vi "query UL_DL Channel Bandwidth.vi"(8 "error in (no error)":errorcluster, 9 "Direction":T1, 10 "Bandwidth Setting Param":T2, 11 "NR in":refnum<class "NR.lvclass">) -> (0 "error out":errorcluster, 2 "BW (MHz)":u32, 3 "NR out":refnum<class "NR.lvclass">)   [LabVIEW 2023, in "ANRITSU Call Box.lvlib" / "NR.lvclass"]
uses:
  NR.lvclass
  NR.lvclass/NR.ctl
  Type Definition/Uplink Downlink Enum.ctl
  ANRITSU Call Box.lvlib
  Type Definition/NR Channel Bandwidth Param.ctl
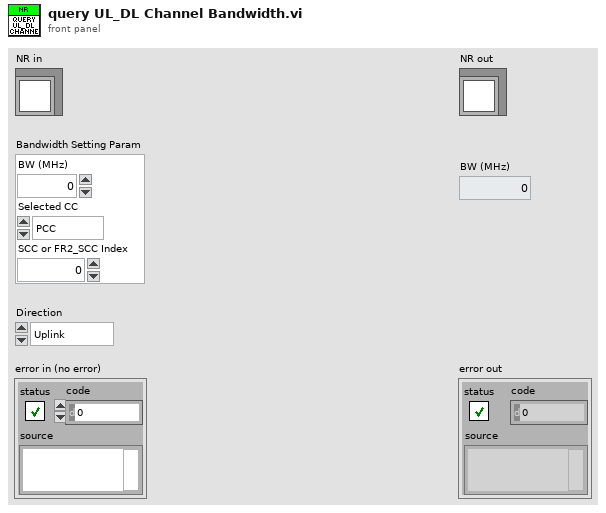
[diagram p1: front panel]
types:
  T1 = typedef "ANRITSU Call Box.lvlib/Uplink Downlink Enum.ctl" = enum16{"Uplink", "Downlink"}
  T2 = typedef "ANRITSU Call Box.lvlib/NR Channel Bandwidth Param.ctl" = cluster{"BW (MHz)":u32, "Selected CC":enum16{"PCC", "SCC", "FR2_PCC", "FR2_SCC"}, "SCC or FR2_SCC Index":u32}
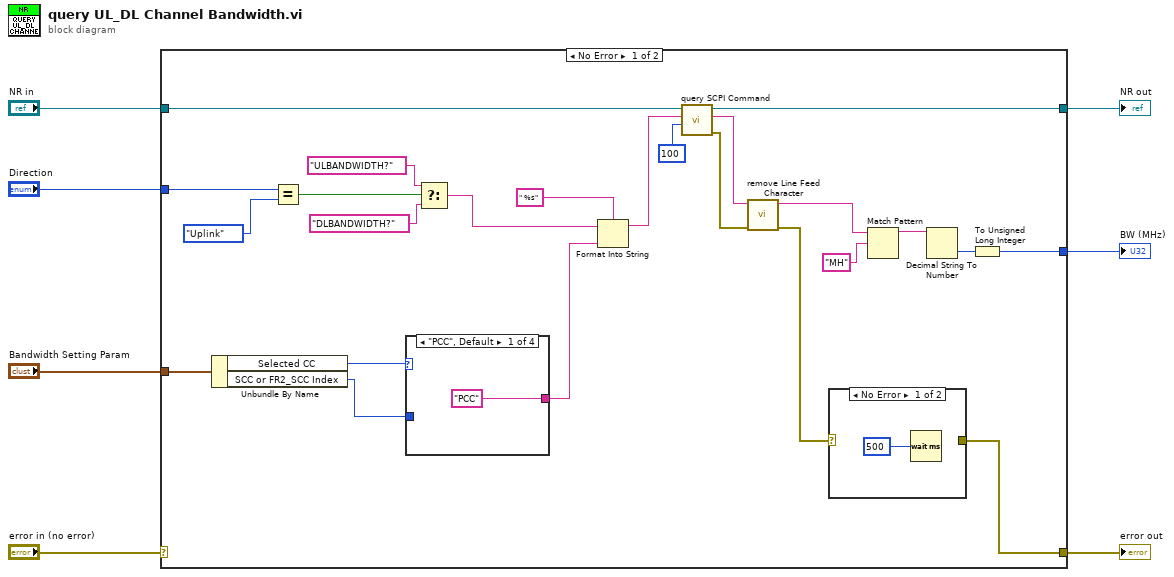
[diagram p0: block diagram]
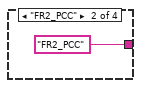
[diagram p3: hidden frame]
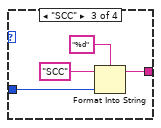
[diagram p4: hidden frame]
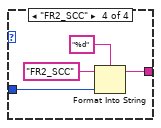
[diagram p5: hidden frame]
diagram:
  n1 = case shown="No Error" "error in (no error)" {
    selector: "error in (no error)" -> [_ w45]
    tunnel: [w21 w45] -> w2
    tunnel: [w10 w44] -> w3
    tunnel: "NR in" -> [w13 w44]
    tunnel: "Direction" -> [w31 _]
    tunnel: "Bandwidth Setting Param" -> [w22 _]
    tunnel: [w14 _] -> w1
    frame No Error {
      n2 = Unbundle By Name(w22) -> ("Selected CC"=w26:enum16{"PCC", "SCC", "FR2_PCC", "FR2_SCC"}, "SCC or FR2_SCC Index"=w25:u32)
      n3 = Equal?(x=w31, y=Uplink_Downlink_Enum."Uplink") -> (x = y?=w27:bool)
      n4 = case shown="\"PCC\", Default" w26 {
        tunnel: ["PCC" "FR2_PCC" w37 w41] -> w23
        tunnel: w25 -> [_ _ w36 w40]
        frame "PCC", Default {
        }
        frame "FR2_PCC" {
        }
        frame "SCC" {
          n5 = Format Into String(format string="%d", initial string="SCC", w36) -> (resulting string=w37:string)  [unwired: 1 in, 1 out]
        }
        frame "FR2_SCC" {
          n6 = Format Into String(format string="%d", initial string="FR2_SCC", w40) -> (resulting string=w41:string)  [unwired: 1 in, 1 out]
        }
      }
      n7 = Select(t="ULBANDWIDTH?" ("format string"), s=w27, f="DLBANDWIDTH?" ("format string")) -> (s? t:f=w24:string)
      n8 = Format Into String(format string=" %s", initial string=w24, w23) -> (resulting string=w12:string)  [unwired: 1 in, 1 out]
      n9 = call "query SCPI Command.vi"("Read Buffer Length"=u32 100, "SCPI Command"=w12, "NR in"=w13) -> ("error out"=w8:errorcluster, "Read Buffer String"=w9:string, "NR out"=w10:refnum<class "NR.lvclass">)  [unwired: 6 in]
      n10 = call "remove Line Feed Character.vi"("error in"=w8, "Query String"=w9) -> ("error out"=w15:errorcluster, "Line Feed Removed String"=w17:string)  [unwired: 8 in]
      n11 = case shown="No Error" w15 {
        selector: w15 -> [_ w33]
        tunnel: [_ w33] -> w21
        frame No Error {
          n12 = Wait (ms)(milliseconds to wait=u32 500) -> ()  [unwired: 1 out]
        }
        frame Error {
        }
      }
      n13 = Match Pattern(string=w17, regular expression="MH") -> (before substring=w19:string)  [unwired: 1 in, 3 out]
      n14 = Decimal String To Number(string=w19) -> (number=w18:i32)  [unwired: 2 in, 1 out]
      n15 = To Unsigned Long Integer(number=w18) -> (unsigned 32bit integer=w14:u32)
    }
    frame Error {
    }
  }
  "error out" <- w2
  "NR out" <- w3
  "BW (MHz)" <- w1
